vi "Array_operation.vi"() -> ()   [LabVIEW 2018]
uses:
  <vilib>/Analysis/Matrix/Datatypes/RealMatrix.ctl
  6bd4d472-6cd2-4c90-b866-ec89ddc20245.vi
  <vilib>/Analysis/Matrix/Numeric/Conversions/Array To Matrix - RA.vi
  <vilib>/Analysis/Matrix/NI_Matrix.lvlib
panel:
  in  "element 5":dbl
  in  "element 4":dbl
  in  "element 3":dbl
  out "appended array":dbl[](array[numeric])
  in  "element 2":dbl
  out "array out":dbl[](array[numeric]) format="%.2f"
  out "Real Matrix (Column Vector)":T1
  out "array (last n elements first)":dbl[](array[numeric])
  out "sorted array":dbl[](array[numeric])
  out "min index(es)":i32
  out "min value":dbl
  out "max index(es)":i32
  out "max value":dbl
  out "output array":dbl[](array[numeric])
  out "element":dbl
  out "size(s)":i32
  in  "Array 5":dbl[](array[numeric])
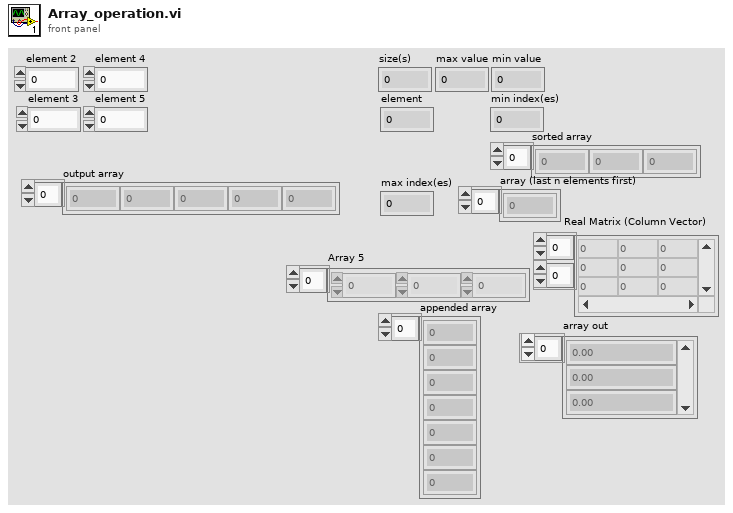
[diagram p1: front panel]
types:
  T1 = typedef "NI_Matrix.lvlib/RealMatrix.ctl" = dbl[][]
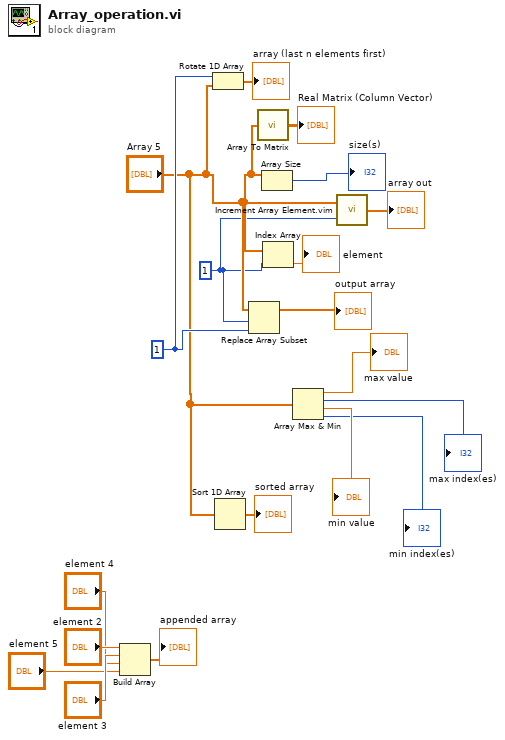
[diagram p0: block diagram]
diagram:
  w11 = 1
  w7 = 1
  n1 = Build Array("element 2", "element 3", "element 4", "element 5") -> (→"appended array":dbl[])
  n2 = Rotate 1D Array(1:"Array 5", 2:w11) -> (0:→"array (last n elements first)":dbl[])
  n3 = Sort 1D Array(array="Array 5") -> (sorted array=→"sorted array":dbl[])
  n4 = Replace Array Subset(array="Array 5", new element=w11, index=w7) -> (→"output array":dbl[])
  n5 = call-poly <vilib>:"Array To Matrix.vi"("Real 1D Array"="Array 5") -> ("Real Matrix (Column Vector)"=→"Real Matrix (Column Vector)":T1)
  n6 = Array Size(array="Array 5") -> (size(s)=→"size(s)":i32)
  n7 = Index Array(array="Array 5", index=w7) -> (element=→"element":dbl)
  n8 = Array Max & Min(array="Array 5") -> (max value=→"max value":dbl, max index (indices)=→"max index(es)":i32, min value=→"min value":dbl, min index (indices)=→"min index(es)":i32)
  n9 = call "Increment Array Element.vim"("index"=w7, "array in"="Array 5") -> ("array out"=→"array out":dbl[])
